vi "stream points to channel.vi"(10 "Points":cluster{"Time Stamp":timestamp, "Value":dbl}[](array[cluster]) {"Time Stamp" format="%<%x %.3X>T"}, 11 "channel":refnum<class "Channel.lvclass">) -> (0 "error out":errorcluster)   [LabVIEW 2020, in "nominal core steps.lvlib"]
doc: "Streams an array of time/value points."
uses:
  nominal core steps.lvlib
  <vilib>/Nominal/Nominal IO Client/submodules/nominal-streaming-labview-ffi/lv_src/Channel/Channel.lvclass
  <vilib>/Nominal/Nominal IO Client/submodules/nominal-streaming-labview-ffi/lv_src/Channel/Push Points Batch_XY.vi
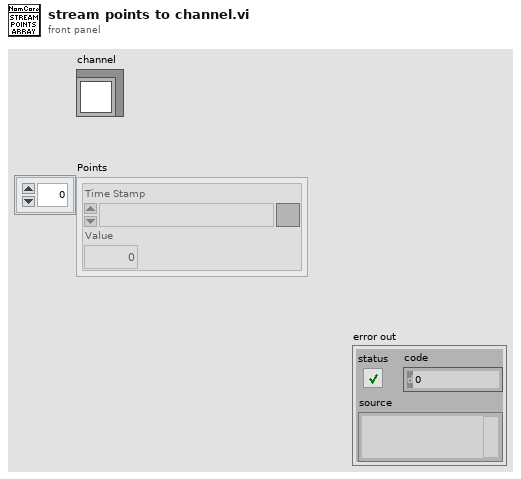
[diagram p1: front panel]
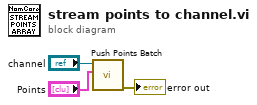
[diagram p0: block diagram]
diagram:
  n1 = call-poly <vilib>:"Push Points Batch.vi"("Points"="Points", "Channel in"="channel") -> ("error out"=→"error out":errorcluster)  [unwired: 8 in, 1 out]
